vi "VIH HelpGen - Image - Search Subset in 2D Array.vi"(6 "Min Row":i32, 8 "Finish Indices":cluster{"Row":i32, "Column":i32}={"Row"=-1, "Column"=-1}, 9 "Start Indices":cluster{"Row":i32, "Column":i32}, 10 "2D subset":u32[][](array[numeric]), 11 "Master 2D array":u32[][](array[numeric])) -> (0 "found":bool, 1 "Found Indices":cluster{"Row":i32, "Column":i32}, 2 "Bounds":cluster{"X0":i32, "Y0":i32, "X1":i32, "Y1":i32})   [LabVIEW 2014]
doc: "::: VI Helpeks :::\nCopyright (c) 2000-2026 Konstantin Shifershteyn. All rights reserved."
panel:
  # "VI Helpeks\nCopyright (c) 2012-2026 Konstantin Shifershteyn"
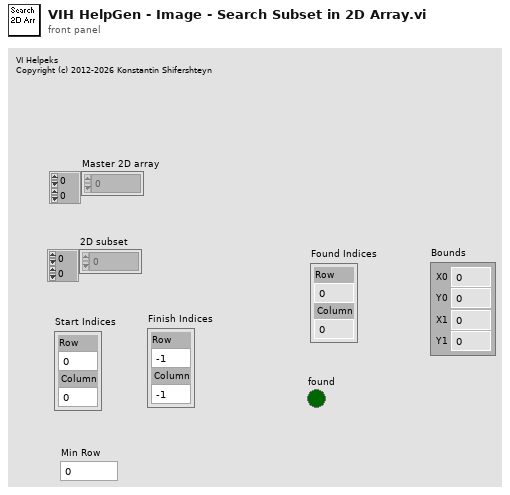
[diagram p1: front panel]
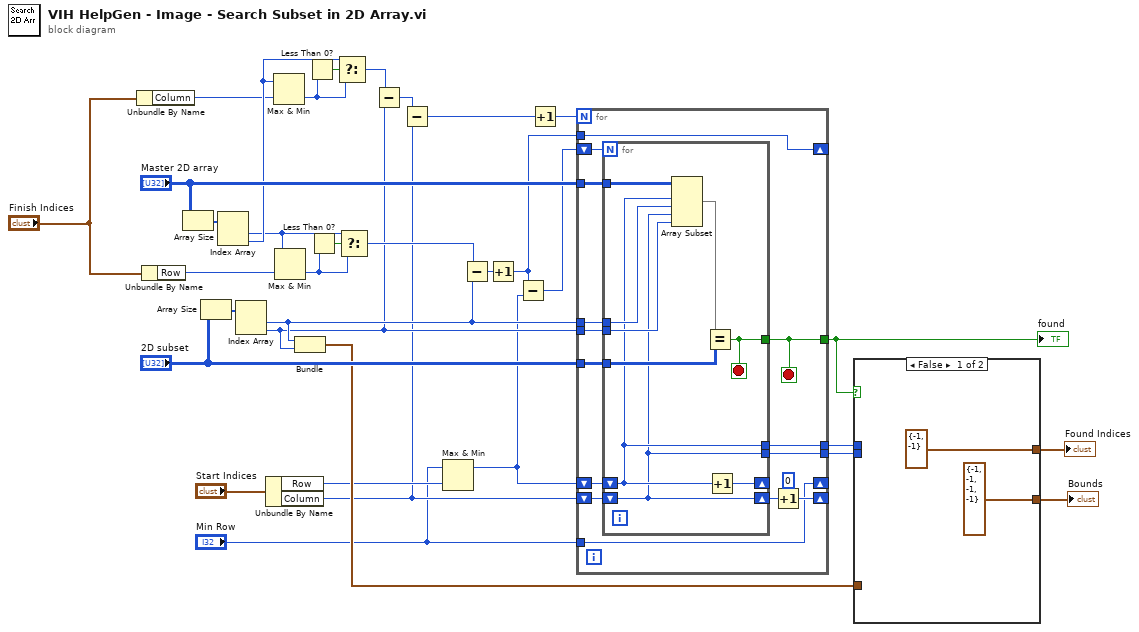
[diagram p0: block diagram]
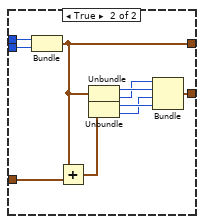
[diagram p2: hidden frame]
diagram:
  n1 = Unbundle By Name("Finish Indices") -> ("Column"=w5:i32)
  n2 = Unbundle By Name("Finish Indices") -> ("Row"=w2:i32)
  n3 = Array Size(array="Master 2D array") -> (size(s)=w32:i32[])
  n4 = Array Size(array="2D subset") -> (size(s)=w34:i32[])
  n5 = Index Array(array=w32) -> (element #1=w1:i32, element #2=w6:i32)  [unwired: 2 in]
  n6 = Index Array(array=w34) -> (element #1=w15:i32, element #2=w14:i32)  [unwired: 2 in]
  n7 = Unbundle By Name("Start Indices") -> ("Row"=w10:i32, "Column"=w8:i32)
  n8 = Max & Min(x=w6, y=w5) -> (min(x,y)=w4:i32)  [unwired: 1 out]
  n9 = Max & Min(x=w1, y=w2) -> (min(x,y)=w3:i32)  [unwired: 1 out]
  n10 = Bundle(w15, w14) -> (w13:cluster{i32, i32})  [unwired: 1 in]
  n11 = Less Than 0?(x=w4) -> (x < 0?=w29:bool)
  n12 = Less Than 0?(x=w3) -> (x < 0?=w23:bool)
  n13 = Select(t=w6, s=w29, f=w4) -> (s? t:f=w28:i32)
  n14 = Select(t=w1, s=w23, f=w3) -> (s? t:f=w24:i32)
  n15 = Subtract(x=w28, y=w14) -> (x-y=w27:i32)
  n16 = Subtract(x=w27, y=w8) -> (x-y=w26:i32)
  n17 = Max & Min(x="Min Row", y=w10) -> (max(x,y)=w9:i32)  [unwired: 1 out]
  n18 = Subtract(x=w24, y=w15) -> (x-y=w25:i32)
  n19 = Increment(x=w25) -> (x+1=w11:i32)
  n20 = Subtract(x=w11, y=w9) -> (x-y=w12:i32)
  n21 = Increment(x=w26) -> (x+1=w19:i32)
  n22 = for {
    N: w19 -> [_]
    shift-right: [w40] -> _
    shift-left: w8 -> [w42]
    tunnel: "Master 2D array" -> [w47]
    tunnel: w15 -> [w46]
    tunnel: w14 -> [w45]
    tunnel: "2D subset" -> [w44]
    tunnel: [w43] -> w18
    tunnel: [w38] -> w21
    tunnel: [w37] -> w20
    shift-right: [w36] -> _
    shift-left: w12 -> [w39]
    tunnel: w11 -> [w36]
    shift-right: [w35] -> _
    shift-left: w9 -> [w48]
    tunnel: "Min Row" -> [w35]
    stop <- w43 stop-if-true
    (unwired) 0 ("Row")
    n23 = for {
      N: w39 -> [_]
      shift-right: [w52] -> _
      shift-left: w48 -> [w50]
      tunnel: w47 -> [w57]
      tunnel: w46 -> [w56]
      tunnel: w45 -> [w55]
      tunnel: w44 -> [w54]
      tunnel: [w51] -> w43
      shift-right: [w49] -> w41
      shift-left: w42 -> [w49]
      tunnel: [w50] -> w38
      tunnel: [w49] -> w37
      stop <- w51 stop-if-true
      n24 = Array Subset(array=w57, index (row)=w50, length (row)=w56, index (col)=w49, length (col)=w55) -> (w53:u32[][])
      n25 = Equal?(x=w53, y=w54) -> (x = y?=w51:bool)
      n26 = Increment(x=w50) -> (x+1=w52:i32)
    }
    n27 = Increment(x=w41) -> (x+1=w40:i32)
  }
  "found" <- w18
  n28 = case shown="False" w18 {
    tunnel: w21 -> [_ w69]
    tunnel: w20 -> [_ w68]
    tunnel: [cluster{"Row":i32, "Column":i32} {"Row"=-1, "Column"=-1} ("f") w63] -> w17
    tunnel: [cluster{"Column":i32, "Row":i32, i32, i32} {"Column"=-1, "Row"=-1, -1, -1} w61] -> w16
    tunnel: w13 -> [_ w60]
    frame False {
    }
    frame True {
      n29 = Bundle(w69, "Column"=w68) -> (w63:cluster{i32, "Column":i32})  [unwired: 1 in]
      n30 = Add(x=w63, y=w60) -> (x+y=w67:cluster{i32, i32})
      n31 = Unbundle(w63) -> (w66:i32, "Column"=w62:i32)
      n32 = Unbundle(w67) -> (w65:i32, w64:i32)
      n33 = Bundle("Column"=w62, w66, w64, w65) -> (w61:cluster{"Column":i32, i32, i32, i32})  [unwired: 1 in]
    }
  }
  "Found Indices" <- w17
  "Bounds" <- w16
